vi "gdi32 SelectObject.vi"(0 "hdc":u64, 5 "h":u64, 11 "error in":errorcluster) -> (4 "previous object":u64, 15 "error out":errorcluster)   [LabVIEW 2020, in "RemoteVI.lvlib"]
doc: "Selects the GDI object h (a bitmap, pen, brush ...) into the device context hdc through gdi32.dll SelectObject (stdcall, called in any thread) and returns the object it replaced - select that one back before deleting h. When error in carries an error the DLL is not called. Generated by scripts\\Build Win32 Wrappers.vi - do not edit by hand, rebuild it."
uses:
  RemoteVI.lvlib
  gdi32.dll
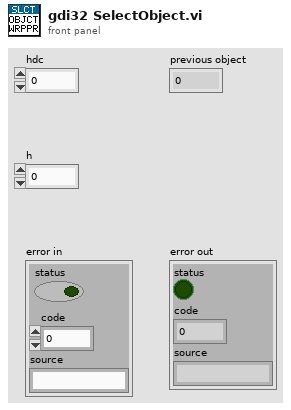
[diagram p1: front panel]
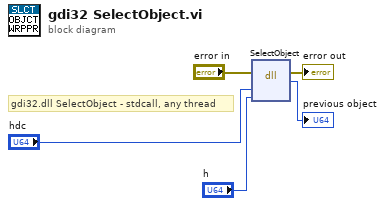
[diagram p0: block diagram]
diagram:
  # "gdi32.dll SelectObject - stdcall, any thread"
  n1 = dll-call lib="gdi32.dll" fn="SelectObject"(error in="error in", "hdc"="hdc", "h"="h") -> (error out=→"error out":errorcluster, →"previous object":u64)  [unwired: 4 in, 1 out]
